vi "AddDependency.vi"(8 "error in (no error)":errorcluster, 9 "Item to depend on":refnum<class "ILabVIEWItem.lvclass">, 11 "CLabVIEWItem in":refnum<class "CLabVIEWItem.lvclass">) -> (0 "error out":errorcluster, 1 "Relationship type":T1, 3 "CLabVIEWItem out":refnum<class "CLabVIEWItem.lvclass">)   [LabVIEW 2020, in "LabVIEWItem.lvlib" / "CLabVIEWItem.lvclass"]
uses:
  CLabVIEWItem.lvclass
  LabVIEWObjectInterfaces/ILabVIEWItem/RelationshipType.ctl
  CLabVIEWItem.lvclass/CLabVIEWItem.ctl
  LabVIEWObjectInterfaces/ILabVIEWItem/ILabVIEWItem.lvclass
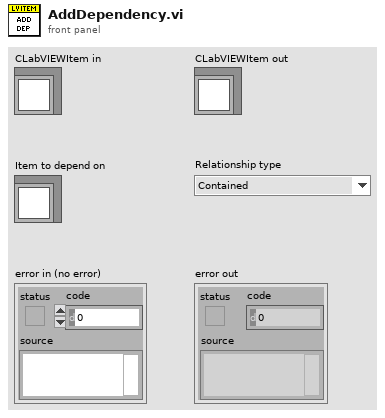
[diagram p1: front panel]
types:
  T1 = typedef "LabVIEWObjectInterfaces.lvlib/ILabVIEWItem.lvclass/RelationshipType.ctl" = enum16{"Contained", "Dependency", "Parent", "Same item", "Related", "None"}
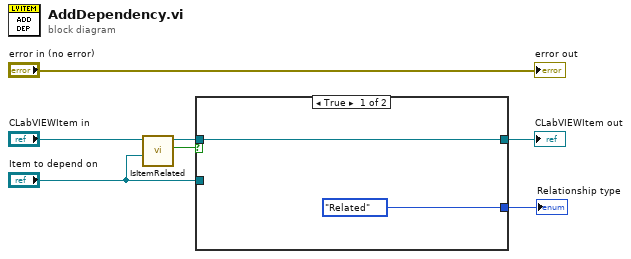
[diagram p0: block diagram]
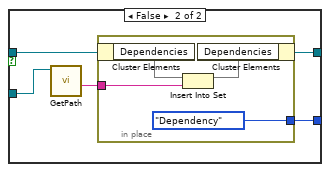
[diagram p2: hidden frame]
diagram:
  n1 = call-dynamic "IsItemRelated.vi"("Item to compare"="Item to depend on", "CLabVIEWItem in"="CLabVIEWItem in") -> ("Is item related?"=w2:bool, "CLabVIEWItem out"=w4:refnum<class "CLabVIEWItem.lvclass">)  [unwired: 7 in, 1 out]
  n2 = case shown="True" w2 {
    tunnel: [w9 w14] -> w7
    tunnel: w4 -> [w9 w13]
    tunnel: "Item to depend on" -> [_ w11]
    tunnel: [RelationshipType."Related" ("Relationship type") w10] -> w1
    frame True {
    }
    frame False {
      n3 = call-dynamic "GetPath.vi"("ILabVIEWItem in"=w11) -> ("Path"=w12:string)  [unwired: 8 in, 2 out]
      n4 = in-place {
        in-place-border: w12 -> [w16]
        in-place-border: [RelationshipType."Dependency" ("Relationship type")] -> w10
        n5 = in-place-cluster #1(w13) -> ("Dependencies"=w18:set{string})
        n6 = Insert Into Set(10:w16, 11:w18) -> (3:w17:set{string})  [unwired: 1 out]
        n7 = in-place-cluster #1("Dependencies"=w17) -> (w14:refnum<class "CLabVIEWItem.lvclass">)
      }
    }
  }
  "CLabVIEWItem out" <- w7
  "Relationship type" <- w1
  "error out" <- "error in (no error)"
